vi "Calculate N_total and Updates.vi"(11 "Generator in":refnum<class "Generator.lvclass">) -> (1 "Updates":i32, 2 "Total Samples":i32, 3 "Samples/Update":i32)   [LabVIEW 2019, in "Generator.lvclass"]
uses:
  Generator.lvclass
  Generator.lvclass/Generator.ctl
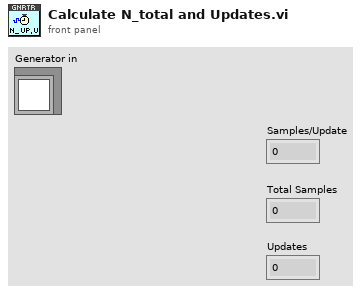
[diagram p1: front panel]
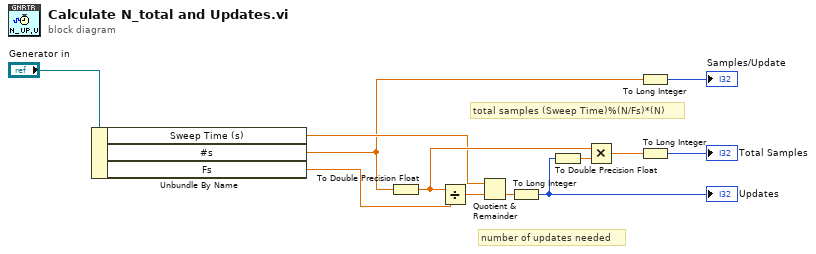
[diagram p0: block diagram]
diagram:
  # "number of updates needed"
  # "total samples (Sweep Time)%(N/Fs)*(N)"
  n1 = Unbundle By Name("Generator in") -> ("Sweep Time (s)"=w3:dbl, "#s"=w2:dbl, "Fs"=w4:dbl)
  n2 = To Double Precision Float(number=w2) -> (double precision float=w8:dbl)
  n3 = Divide(x=w8, y=w4) -> (x/y=w9:dbl)
  n4 = Quotient & Remainder(x=w3, y=w9) -> (floor(x/y)=w10:dbl)  [unwired: 1 out]
  n5 = To Long Integer(number=w10) -> (32bit integer=w11:i32)
  "Updates" <- w11
  n6 = To Double Precision Float(number=w11) -> (double precision float=w6:dbl)
  n7 = Multiply(x=w8, y=w6) -> (x*y=w12:dbl)
  n8 = To Long Integer(number=w2) -> (32bit integer=→"Samples/Update":i32)
  n9 = To Long Integer(number=w12) -> (32bit integer=→"Total Samples":i32)
